vi "SDO_TRAJECTORY_EXECUTE_ABS.vi"(8 "Init":bool, 11 "End Pose ENG":T1={"TRANSLATION"={"X"=0.0, "Y"=0.0}, "ROTATION"={"VALUE"=0.0, "COS"=1.0, "SIN"=0.0}} {"ROTATION"."SIN" format="%13.4f"; "ROTATION"."COS" format="%13.4f"; "ROTATION"."VALUE" format="%13.4f"; "TRANSLATION"."Y" format="%14.3f"; "TRANSLATION"."X" format="%14.3f"}) -> (0 "AtReference":bool, 3 "Chassis Velocity Target":T4 {"vOmega" format="%10.3f"; "vY" format="%10.3f"; "vX" format="%10.3f"})   [LabVIEW 2019]
uses:
  <vilib>/Rock Robotics/WPI/ThirdParty/JAS_Junk/TrajLib/TypeDef/CHASSIS_SPEEDS.ctl
  <vilib>/Rock Robotics/WPI/ThirdParty/JAS_Junk/TrajLib/TypeDef/POSE2D.ctl
  <vilib>/Rock Robotics/WPI/ThirdParty/JAS_Junk/TrajLib/TypeDef/TRANSLATION2D.ctl
  <vilib>/Rock Robotics/WPI/ThirdParty/JAS_Junk/TrajLib/TypeDef/ROTATION2D.ctl
  <vilib>/Rock Robotics/WPI/ThirdParty/JAS_Junk/TrajLib/VI/Util_GetTime_U32.vi
  <vilib>/Rock Robotics/WPI/ThirdParty/JAS_Junk/TrajLib/ProfiledPIDController_NewPeriod.vi
  <vilib>/Rock Robotics/WPI/ThirdParty/JAS_Junk/TrajLib/ProfiledPIDController_SetIntegratorRange.vi
  <vilib>/Rock Robotics/WPI/ThirdParty/JAS_Junk/TrajLib/ProfiledPIDController_DisableContInput.vi
  <vilib>/Rock Robotics/WPI/ThirdParty/JAS_Junk/TrajLib/ProfiledPIDController_EnableContInput.vi
  <vilib>/Rock Robotics/WPI/ThirdParty/JAS_Junk/TrajLib/TrapProfConstraint_New.vi
  <vilib>/Rock Robotics/WPI/ThirdParty/JAS_Junk/TrajLib/HolDrvCtrl_New.vi
  <vilib>/Rock Robotics/WPI/ThirdParty/JAS_Junk/TrajLib/HolDrvCtrl_PackPID.vi
  <vilib>/Rock Robotics/WPI/ThirdParty/JAS_Junk/TrajLib/HolDrvCtrl_SetTolerance.vi
  <vilib>/Rock Robotics/WPI/ThirdParty/JAS_Junk/TrajLib/HolDrvCtrl_SetEnabled.vi
  <vilib>/Rock Robotics/WPI/ThirdParty/JAS_Junk/TrajLib/HolDrvCtrl_Calculate_Trajectory.vi
  <vilib>/Rock Robotics/WPI/ThirdParty/JAS_Junk/TrajLib/HolDrvCtrl_AtReference.vi
  <vilib>/Rock Robotics/WPI/ThirdParty/JAS_Junk/TrajLib/TrapProfState_New.vi
  <vilib>/Rock Robotics/WPI/ThirdParty/JAS_Junk/TrajLib/PIDController_NewPeriod.vi
  <vilib>/Rock Robotics/SystemInterfaces/NetworkCommunication/NetComm_UsageReport_report.vi
  <vilib>/Rock Robotics/WPI/ThirdParty/JAS_Junk/TrajLib/PIDController_SetIntegratorRange.vi
  <vilib>/Rock Robotics/WPI/ThirdParty/JAS_Junk/TrajLib/PIDController_DisableContinousInput.vi
  <vilib>/Rock Robotics/WPI/ThirdParty/JAS_Junk/TrajLib/PIDController_EnableContinousInput.vi
  <vilib>/Rock Robotics/WPI/ThirdParty/JAS_Junk/TrajLib/Conv_Deg_Radians.vi
  <vilib>/Rock Robotics/WPI/ThirdParty/JAS_Junk/TrajLib/PIDController_Reset.vi
  <vilib>/Rock Robotics/WPI/ThirdParty/JAS_Junk/TrajLib/HolDrvCtrl_Calculate.vi
  <vilib>/Rock Robotics/WPI/ThirdParty/JAS_Junk/TrajLib/Rotation2d_GetRadians.vi
  <vilib>/Rock Robotics/WPI/ThirdParty/JAS_Junk/TrajLib/Rotation2d_GetAngleCosSin.vi
  <vilib>/Rock Robotics/WPI/ThirdParty/JAS_Junk/TrajLib/Pose2d_RelativeTo.vi
  <vilib>/Rock Robotics/WPI/ThirdParty/JAS_Junk/TrajLib/Pose2d_getRotation.vi
  <vilib>/Rock Robotics/WPI/ThirdParty/JAS_Junk/TrajLib/Rotation2d_Minus.vi
  <vilib>/Rock Robotics/WPI/ThirdParty/JAS_Junk/TrajLib/ProfiledPIDController_Calculate_Meas_Goal.vi
  <vilib>/Rock Robotics/WPI/ThirdParty/JAS_Junk/TrajLib/PIDController_Calculate_SP_PV.vi
  <vilib>/Rock Robotics/WPI/ThirdParty/JAS_Junk/TrajLib/ProfiledPIDController_Reset_PosOnly.vi
  <vilib>/Rock Robotics/WPI/ThirdParty/JAS_Junk/TrajLib/ChassisSpeeds_FromFieldRelativeSpeeds.vi
  <vilib>/Rock Robotics/WPI/ThirdParty/JAS_Junk/TrajLib/Transform2d_Create_PosePose.vi
  <vilib>/Rock Robotics/WPI/ThirdParty/JAS_Junk/TrajLib/Pose2d_New_TRRO.vi
  <vilib>/Rock Robotics/WPI/ThirdParty/JAS_Junk/TrajLib/Rotation2d_UnaryMinus.vi
  <vilib>/Rock Robotics/WPI/ThirdParty/JAS_Junk/TrajLib/Rotation2d_RotateBy.vi
  <vilib>/Rock Robotics/WPI/ThirdParty/JAS_Junk/TrajLib/ProfiledPIDController_SetGoal_PosOnly.vi
  <vilib>/Rock Robotics/WPI/ThirdParty/JAS_Junk/TrajLib/ProfiledPIDController_Calculate_Meas.vi
  <vilib>/Rock Robotics/WPI/ThirdParty/JAS_Junk/TrajLib/PIDController_SetSetpoint.vi
  <vilib>/Rock Robotics/WPI/ThirdParty/JAS_Junk/TrajLib/PIDController_Calculate_PV.vi
  <vilib>/Rock Robotics/WPI/ThirdParty/JAS_Junk/TrajLib/ProfiledPIDController_Reset.vi
  <vilib>/Rock Robotics/WPI/ThirdParty/JAS_Junk/TrajLib/Rotation2d_GetCos.vi
  <vilib>/Rock Robotics/WPI/ThirdParty/JAS_Junk/TrajLib/Rotation2d_GetSin.vi
  <vilib>/Rock Robotics/WPI/ThirdParty/JAS_Junk/TrajLib/Translation2d_RotateBy.vi
  <vilib>/Rock Robotics/WPI/ThirdParty/JAS_Junk/TrajLib/Translation2d_Minus.vi
  <vilib>/Rock Robotics/WPI/ThirdParty/JAS_Junk/TrajLib/Rotation2d_CreateAngle.vi
  <vilib>/Rock Robotics/WPI/ThirdParty/JAS_Junk/TrajLib/Rotation2d_CreateXY.vi
  <vilib>/Rock Robotics/WPI/ThirdParty/JAS_Junk/TrajLib/ProfiledPIDController_SetGoal.vi
  <vilib>/Rock Robotics/WPI/ThirdParty/JAS_Junk/TrajLib/TrapProfile_New.vi
  <vilib>/Rock Robotics/WPI/ThirdParty/JAS_Junk/TrajLib/ProfiledPIDController_GetPeriod.vi
  <vilib>/Rock Robotics/WPI/ThirdParty/JAS_Junk/TrajLib/TrapProfile_Calculate.vi
  <vilib>/Rock Robotics/WPI/ThirdParty/JAS_Junk/TrajLib/ControllerUtil_GetModulusError.vi
  <vilib>/Rock Robotics/WPI/ThirdParty/JAS_Junk/TrajLib/Translation2d_Create.vi
  <vilib>/Rock Robotics/WPI/ThirdParty/JAS_Junk/TrajLib/Util_CalcDist.vi
  <vilib>/Rock Robotics/WPI/ThirdParty/JAS_Junk/TrajLib/TrapProfile_ShouldFlipAcceleration.vi
  <vilib>/Rock Robotics/WPI/ThirdParty/JAS_Junk/TrajLib/TrapProfile_Direct.vi
  <vilib>/Rock Robotics/WPI/ThirdParty/JAS_Junk/TrajLib/PIDController_GetPeriod.vi
  <vilib>/Rock Robotics/WPI/ThirdParty/JAS_Junk/TrajLib/VI/Util_GetTime_U64.vi
  SDO_TRAJECTORY_GLOBALS.vi
  <vilib>/Rock Robotics/WPI/ThirdParty/JAS_Junk/TrajLib/Globals/Util_LibraryGlobals.vi
  Swerve_Drive_System/SDO_DRIVE_GLOBALS.vi
  <vilib>/Rock Robotics/WPI/ThirdParty/JAS_Junk/TrajLib/Trajectory_Library.lvlib
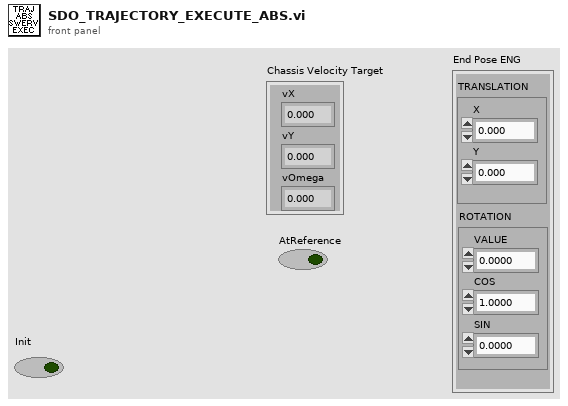
[diagram p1: front panel]
types:
  T1 = typedef "Trajectory_Library.lvlib/POSE2D.ctl" = cluster{"TRANSLATION":T2, "ROTATION":T3}
  T2 = typedef "Trajectory_Library.lvlib/TRANSLATION2D.ctl" = cluster{"X":dbl, "Y":dbl}
  T3 = typedef "Trajectory_Library.lvlib/ROTATION2D.ctl" = cluster{"VALUE":dbl, "COS":dbl, "SIN":dbl}
  T4 = typedef "Trajectory_Library.lvlib/CHASSIS_SPEEDS.ctl" = cluster{"vX":dbl, "vY":dbl, "vOmega":dbl}
  T5 = typedef "Trajectory_Library.lvlib/SWERVE_DRIVE_KINEMATICS.ctl" = cluster{"NumModules":i32, "InverseKinematics":T6, "ForwardKinematics":T6, "Modules":T2[], "PrevCoR":T2, "SavedModuleStates":T7[]}
  T6 = typedef "NI_Matrix.lvlib/RealMatrix.ctl" = dbl[][]
  T7 = typedef "Trajectory_Library.lvlib/SWERVE_DRIVE_MODULE_STATE.ctl" = cluster{"Speed":dbl, "Angle":T3}
  T8 = typedef "Trajectory_Library.lvlib/TRAJECTORY.ctl" = cluster{"TotalTImeSecs":dbl, "States":T9[]}
  T9 = typedef "Trajectory_Library.lvlib/TRAJ_STATE.ctl" = cluster{"TimeSeconds":dbl, "Velocity":dbl, "Acceleration":dbl, "POSE":T1, "Curvature":dbl}
  T10 = typedef "Trajectory_Library.lvlib/PID_TUNING.ctl" = cluster{"Kp":dbl, "Ki":dbl, "Kd":dbl, "MaximumIntegral":dbl, "MinimumIntegral":dbl, "IntegralZone":dbl}
  T11 = typedef "Trajectory_Library.lvlib/PROFILED_PID_CONTROLLER.ctl" = cluster{"Controller":T12, "Goal":T13, "Setpoint":T13, "Constraint":T14}
  T12 = typedef "Trajectory_Library.lvlib/PID_CONTROLLER.ctl" = cluster{"Kp":dbl, "Ki":dbl, "Kd":dbl, "Period":dbl, "Max_Integral":dbl, "Min_Integral":dbl, "Max_Input":dbl, "Min_Input":dbl, "Continuous":bool, "PositionError":dbl, "VelocityError":dbl, "PrevError":dbl, "Total_Integral":dbl, "PositionTolerance":dbl, "VelocityTolerance":dbl, "SetPoint":dbl, "Kf":dbl, "Prev_Deriv":dbl, "Prev_Deriv 2":dbl, "DerivativeFilter":bool, "Min_Output":dbl, "Max_Output":dbl, "Prev_F_P":dbl, "Prev_F_P_2":dbl, "AntiWindupActive":bool, "Measurement":dbl, "IntegralZone":dbl}
  T13 = typedef "Trajectory_Library.lvlib/TRAPEZOID_PROFILE_STATE.ctl" = cluster{"Position":dbl, "Velocity":dbl}
  T14 = typedef "Trajectory_Library.lvlib/TRAPEZOID_PROFILE_CONSTRAINT.ctl" = cluster{"MaxVelocity":dbl, "MaxAcceleration":dbl}
  T15 = typedef "Trajectory_Library.lvlib/HOLONOMIC_PACK_TUNING.ctl" = cluster{"X PID Tuning":T10, "Y PID Tuning":T10, "thetaProfiledPID_CTRL":T11}
  T16 = typedef "Trajectory_Library.lvlib/HOLONOMIC_DRV_CTRL.ctl" = cluster{"poseTolerance":T1, "poseError":T1, "Enabled":bool, "PID_xCtrl":T12, "PID_yCtrl":T12, "PROF_PID_thetaCtrl":T11, "RotationError":T3, "FirstRun":bool}
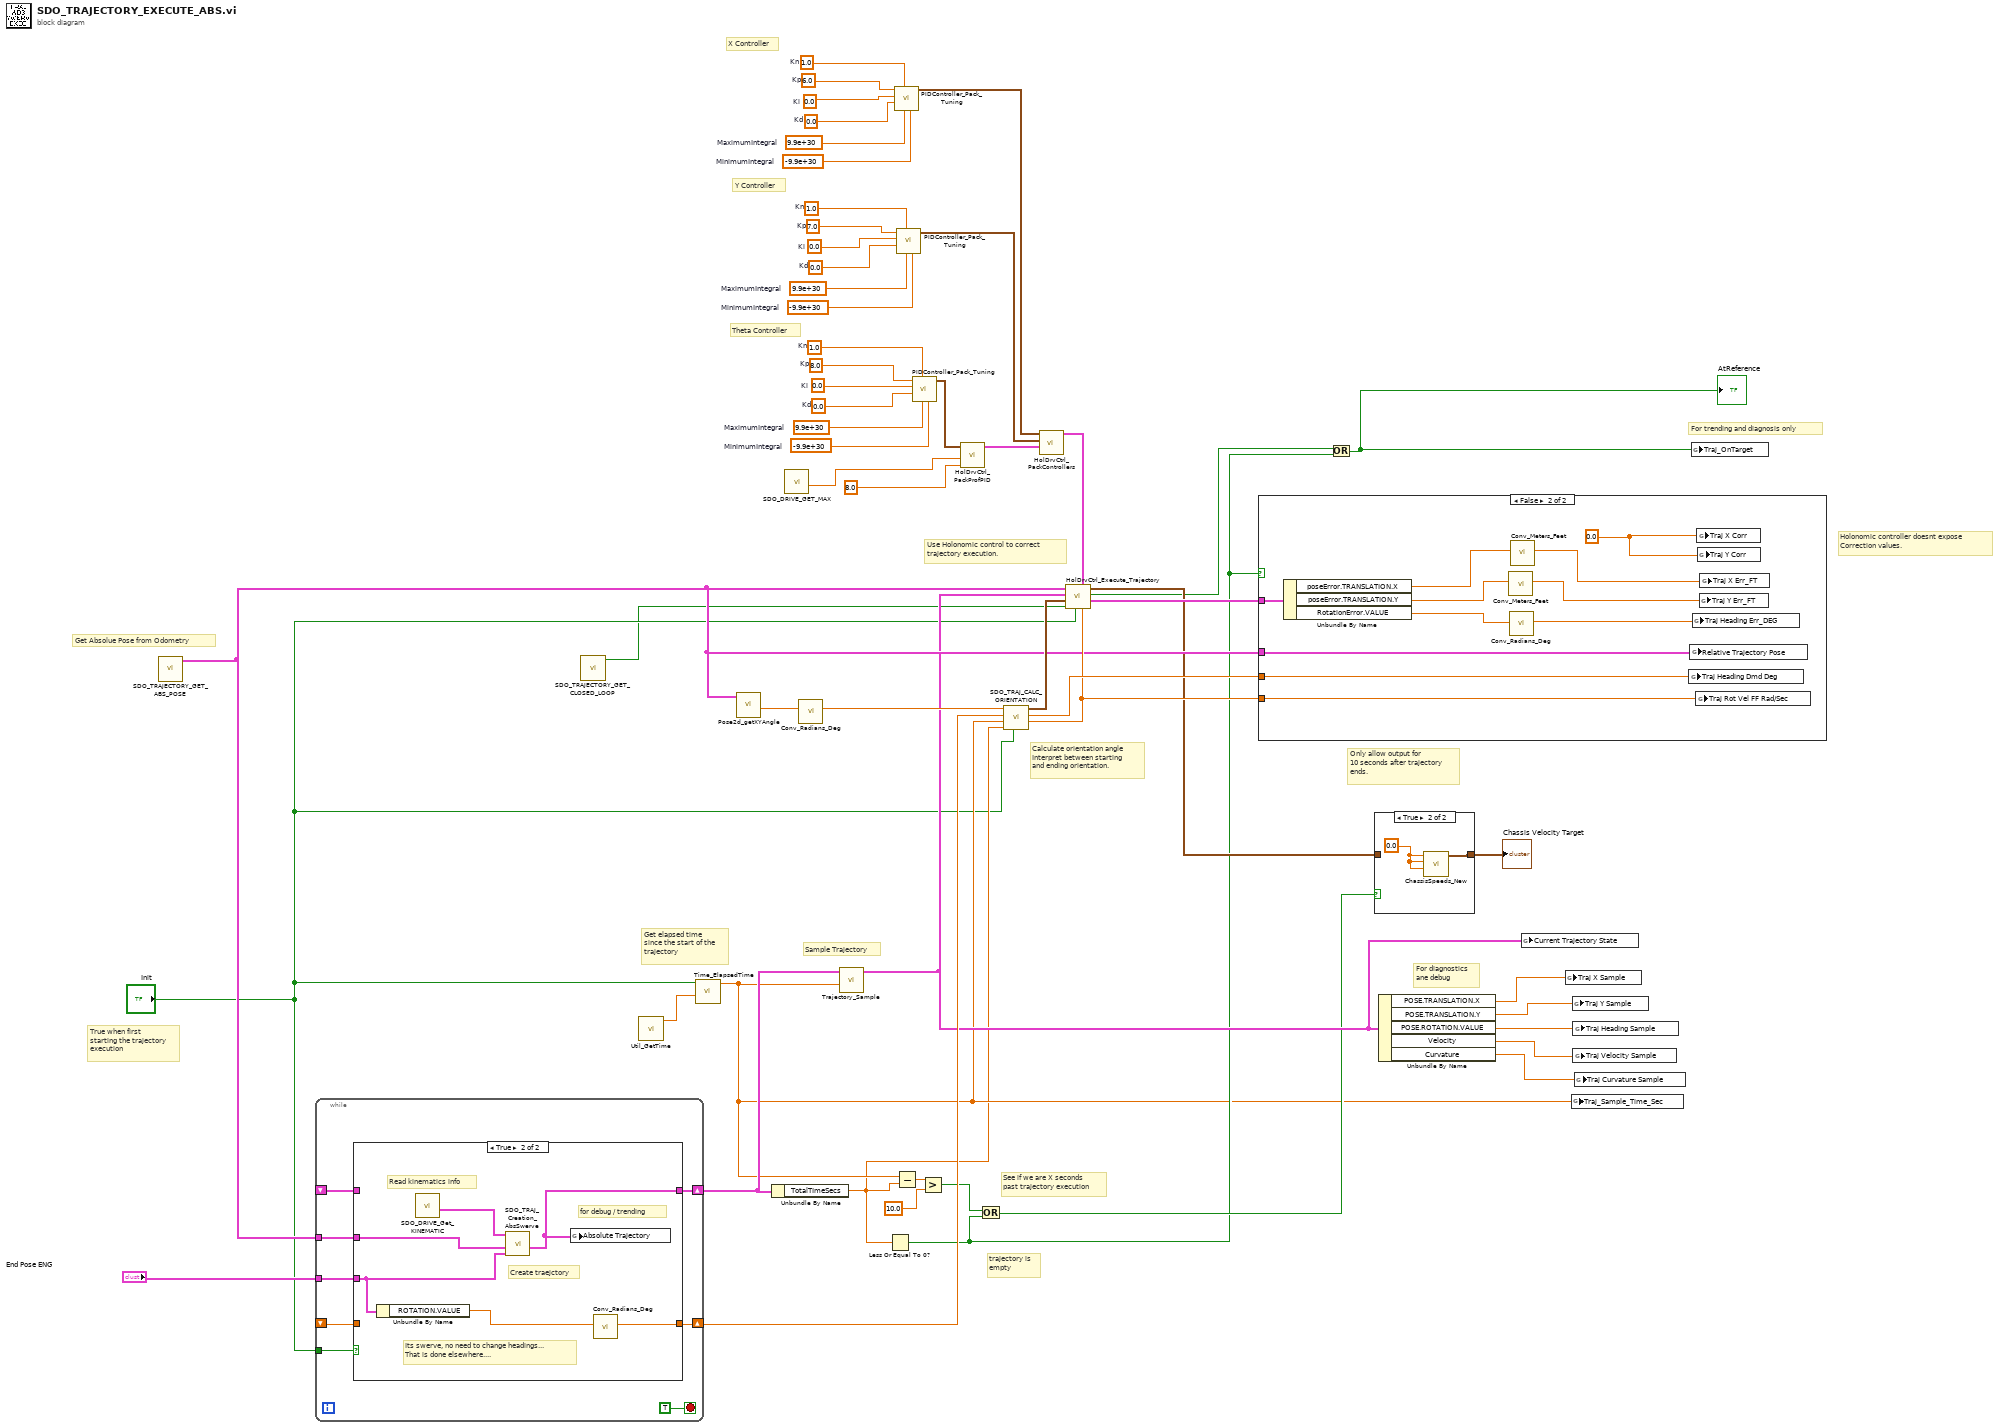
[diagram p0: block diagram]
diagram:
  w26 = 1.0  # Kn
  w29 = 8.0  # Kp
  w38 = 0.0  # Ki
  w39 = 0.0  # Kd
  w40 = 9.9e+30  # MaximumIntegral
  w41 = -9.9e+30  # MinimumIntegral
  w24 = 1.0  # Kn
  w27 = 6.0  # Kp
  w30 = 0.0  # Ki
  w31 = 0.0  # Kd
  w32 = 9.9e+30  # MaximumIntegral
  w33 = -9.9e+30  # MinimumIntegral
  w25 = 1.0  # Kn
  w28 = 7.0  # Kp
  w34 = 0.0  # Ki
  w35 = 0.0  # Kd
  w36 = 9.9e+30  # MaximumIntegral
  w37 = -9.9e+30  # MinimumIntegral
  # "trajectory is \nempty"
  # "Theta Controller"
  # "Y Controller"
  # "X Controller"
  # "Calculate orientation angle\nInterpret between starting\nand ending orientation."
  # "True when first\nstarting the trajectory\nexecution"
  # "Get elapsed time\nsince the start of the\ntrajectory"
  # "Holonomic controller doesnt expose\nCorrection values."
  # "Use Holonomic control to correct\ntrajectory execution."
  # "For trending and diagnosis only"
  # "For diagnostics\nane debug"
  # "Get Absolue Pose from Odometry"
  # "Sample Trajectory"
  # "See if we are X seconds \npast trajectory execution"
  # "Only allow output for\n10 seconds after trajectory\nends."
  n1 = call "SDO_TRAJECTORY_GET_ABS_POSE.vi"() -> ("Absolute Odometry Pose"=w16:T1)  [unwired: 11 in]
  n2 = while {
    tunnel: "Init" -> [w62]
    tunnel: w16 -> [w61]
    shift-right: [w60] -> w17
    shift-left: _ -> [w59]
    shift-right: [w58] -> w13
    shift-left: _ -> [w57]
    tunnel: "End Pose ENG" -> [w56]
    stop <- TRUE stop-if-true
    n3 = case shown="True" w62 {
      tunnel: w61 -> [_ w67]
      tunnel: [w65 w68] -> w60
      tunnel: w59 -> [w65 _]
      tunnel: [w64 w70] -> w58
      tunnel: w57 -> [w64 _]
      tunnel: w56 -> [_ w71]
      frame False {
      }
      frame True {
        # "for debug / trending"
        # "Read kinematics info"
        # "Its swerve, no need to change headings...\nThat is done elsewhere...."
        # "Create traejctory"
        n4 = Unbundle By Name(w71) -> ("ROTATION.VALUE"=w69:dbl)
        n5 = call "SDO_DRIVE_Get_KINEMATIC.vi"() -> ("out SWERVE_DRIVE_KINEMATICS"=w66:T5)  [unwired: 11 in]
        n6 = call "SDO_TRAJ_Creation_AbsSwerve.vi"("End Pose  ENG"=w71, "Current Pose SI"=w67, "SWERVE_DRIVE_KINEMATICS"=w66) -> ("Absolute Trajectory"=w68:T8)  [unwired: 6 in, 2 out]
        n7 = global write "SDO_TRAJECTORY_GLOBALS.vi" "Absolute Trajectory"(w68) -> ()
        n8 = call <vilib>:"Conv_Radians_Deg.vi"("Radians"=w69) -> ("Degrees"=w70:dbl)  [unwired: 10 in]
      }
    }
  }
  n9 = call "SDO_TRAJECTORY_GET_CLOSED_LOOP.vi"() -> ("AUTO_CLOSED_LOOP"=w1:bool)  [unwired: 11 in]
  n10 = call <vilib>:"Util_GetTime.vi"() -> ("FPGA_Time_Seconds"=w52:dbl)  [unwired: 9 in, 2 out]
  n11 = call <vilib>:"Time_ElapsedTime.vi"("PassthroughTime_SEC"=w52, "Reset"="Init") -> ("Elapsed Time Sec"=w4:dbl)  [unwired: 9 in]
  n12 = call <vilib>:"Pose2d_getXYAngle.vi"("in POSE"=w16) -> ("Angle"=w15:dbl)  [unwired: 8 in, 2 out]
  n13 = Unbundle By Name(w17) -> ("TotalTImeSecs"=w3:dbl)
  n14 = call "SDO_DRIVE_GET_MAX.vi"() -> ("Max Rotational Vel (Rad/Sec)"=w19:dbl)  [unwired: 10 in, 1 out]
  n15 = call <vilib>:"Conv_Radians_Deg.vi"("Radians"=w15) -> ("Degrees"=w14:dbl)  [unwired: 10 in]
  n16 = call <vilib>:"Trajectory_Sample.vi"("Time"=w4, "InputTRAJECTORY"=w17) -> ("OutputTRAJ_STATE"=w12:T9)  [unwired: 9 in]
  n17 = Less Or Equal To 0?(x=w3) -> (x <= 0?=w5:bool)
  n18 = call <vilib>:"PIDController_Pack_Tuning.vi"("MinimumIntegral"=w33, "MaximumIntegral"=w32, "Kn"=w24, "Kd"=w31, "Ki"=w30, "Kp"=w27) -> ("PID Tuning"=w42:T10)  [unwired: 5 in]
  n19 = Subtract(x=w4, y=w3) -> (x-y=w55:dbl)
  n20 = call <vilib>:"PIDController_Pack_Tuning.vi"("MinimumIntegral"=w37, "MaximumIntegral"=w36, "Kn"=w25, "Kd"=w35, "Ki"=w34, "Kp"=w28) -> ("PID Tuning"=w43:T10)  [unwired: 5 in]
  n21 = call <vilib>:"PIDController_Pack_Tuning.vi"("MinimumIntegral"=w41, "MaximumIntegral"=w40, "Kn"=w26, "Kd"=w39, "Ki"=w38, "Kp"=w29) -> ("PID Tuning"=w23:T10)  [unwired: 5 in]
  n22 = Greater?(x=w55, y=10.0) -> (0:w9:bool)
  n23 = call <vilib>:"HolDrvCtrl_PackProfPID.vi"("Max Accel"=8.0, "Max Speed"=w19, "Theta PID Tuning"=w23) -> ("Theta PID CONTROLLER"=w44:T11)  [unwired: 8 in]
  n24 = Or(x=w9, y=w5) -> (x .or. y?=w8:bool)
  n25 = call "SDO_TRAJ_CALC_ORIENTATION.vi"("Init"="Init", "Total Trajectory Time Sec"=w3, "Elapsed Traj Time Sec"=w4, "End Orientation Demand DEG"=w13, "Starting Orientation  DEG"=w14) -> ("Rotational Velocity Rad Per Sec"=w20:dbl, "Orientation Demand Deg"=w46:dbl, "Orientation Demand"=w22:T3)  [unwired: 4 in]
  n26 = call <vilib>:"HolDrvCtrl_PackControllers.vi"("thetaProfiledPID_CTRL"=w44, "Y PID Tuning"=w43, "X PID Tuning"=w42) -> ("HOLONOMIC_CTRL_PACK_TUNING"=w45:T15)  [unwired: 8 in]
  n27 = call <vilib>:"HolDrvCtrl_Execute_Trajectory.vi"("Rotational Velocity Feedforward \nRad/Sec"=w20, "HOLONOMIC_CTRL_PACK_TUNING"=w45, "Reset"="Init", "Enable"=w1, "angleRef"=w22, "desiredTrajState"=w12, "currentPose"=w16) -> ("outHOLONOMIC_DRV_CTRL"=w21:T16, "AtReference"=w7:bool, "calcChassisSpeed"=w10:T4)  [unwired: 2 in]
  n28 = case shown="False" w5 {
    tunnel: w46 -> [_ w81]
    tunnel: w21 -> [_ w75]
    tunnel: w20 -> [_ w74]
    tunnel: w16 -> [_ w72]
    frame True {
    }
    frame False {
      w82 = 0.0 ("Y Corr")
      n29 = Unbundle By Name(w75) -> ("poseError.TRANSLATION.X"=w79:dbl, "poseError.TRANSLATION.Y"=w78:dbl, "RotationError.VALUE"=w73:dbl)
      n30 = call <vilib>:"Conv_Meters_Feet.vi"("Meters"=w78) -> ("Feet"=w77:dbl)  [unwired: 10 in]
      n31 = call <vilib>:"Conv_Radians_Deg.vi"("Radians"=w73) -> ("Degrees"=w80:dbl)  [unwired: 10 in]
      n32 = call <vilib>:"Conv_Meters_Feet.vi"("Meters"=w79) -> ("Feet"=w76:dbl)  [unwired: 10 in]
      n33 = global write "SDO_TRAJECTORY_GLOBALS.vi" "Traj Heading Dmd Deg"(w81) -> ()
      n34 = global write "SDO_TRAJECTORY_GLOBALS.vi" "Relative Trajectory Pose"(w72) -> ()
      n35 = global write "SDO_TRAJECTORY_GLOBALS.vi" "Traj Heading Err_DEG"(w80) -> ()
      n36 = global write "SDO_TRAJECTORY_GLOBALS.vi" "Traj Rot Vel FF Rad/Sec"(w74) -> ()
      n37 = global write "SDO_TRAJECTORY_GLOBALS.vi" "Traj X Corr"(w82) -> ()
      n38 = global write "SDO_TRAJECTORY_GLOBALS.vi" "Traj Y Corr"(w82) -> ()
      n39 = global write "SDO_TRAJECTORY_GLOBALS.vi" "Traj Y Err_FT"(w77) -> ()
      n40 = global write "SDO_TRAJECTORY_GLOBALS.vi" "Traj X Err_FT"(w76) -> ()
    }
  }
  n41 = Or(x=w7, y=w5) -> (x .or. y?=w6:bool)
  "AtReference" <- w6
  n42 = case shown="True" w8 {
    tunnel: w10 -> [w83 _]
    tunnel: [w83 w84] -> w53
    frame False {
    }
    frame True {
      w85 = 0.0 ("vX")
      n43 = call <vilib>:"ChassisSpeeds_New.vi"("vAngular"=w85, "vY"=w85, "vX"=w85) -> ("CHASSIS"=w84:T4)  [unwired: 8 in]
    }
  }
  "Chassis Velocity Target" <- w53
  n44 = Unbundle By Name(w12) -> ("POSE.TRANSLATION.X"=w51:dbl, "POSE.TRANSLATION.Y"=w50:dbl, "POSE.ROTATION.VALUE"=w49:dbl, "Velocity"=w48:dbl, "Curvature"=w47:dbl)
  n45 = global write "SDO_TRAJECTORY_GLOBALS.vi" "Current Trajectory State"(w12) -> ()
  n46 = global write "SDO_TRAJECTORY_GLOBALS.vi" "Traj X Sample"(w51) -> ()
  n47 = global write "SDO_TRAJECTORY_GLOBALS.vi" "Traj_Sample_Time_Sec"(w4) -> ()
  n48 = global write "SDO_TRAJECTORY_GLOBALS.vi" "Traj Y Sample"(w50) -> ()
  n49 = global write "SDO_TRAJECTORY_GLOBALS.vi" "Traj Heading Sample"(w49) -> ()
  n50 = global write "SDO_TRAJECTORY_GLOBALS.vi" "Traj Velocity Sample"(w48) -> ()
  n51 = global write "SDO_TRAJECTORY_GLOBALS.vi" "Traj Curvature Sample"(w47) -> ()
  n52 = global write "SDO_TRAJECTORY_GLOBALS.vi" "Traj_OnTarget"(w6) -> ()
